vi "DAC Run.vi"(8 "error in":errorcluster, 11 "DAC HS Vib in":refnum<class "DAC HS Vib.lvclass">) -> (0 "error out":errorcluster, 3 "DAC HS Vib out":refnum<class "DAC HS Vib.lvclass">)   [LabVIEW 2019, in "DAC.lvlib" / "DAC HS Vib.lvclass"]
uses:
  DAC HS Vib.lvclass
  C:/Users/krio/Documents/LV_Projects/test-stand/App/DAC/DAC.lvclass
  DAC.lvclass/DAC.ctl
  DAC.lvclass
  Results/Results Method.ctl
  Results/Results.lvlib
  Results/DeepU Results/DeepU Results.lvclass
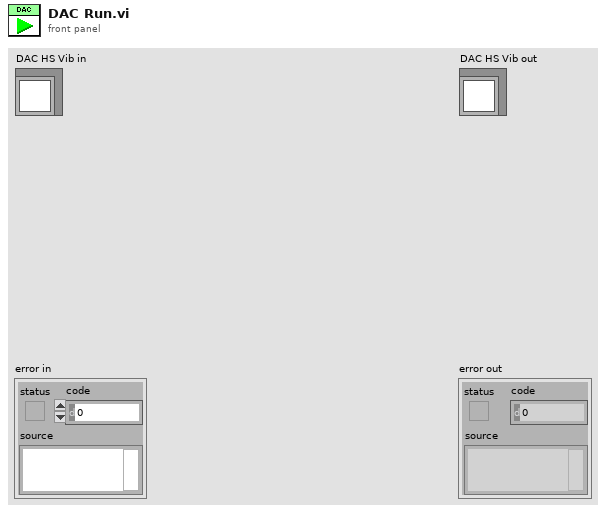
[diagram p1: front panel]
types:
  T1 = typedef "Results.lvlib/Results Method.ctl" = enum16{"Get", "Set"}
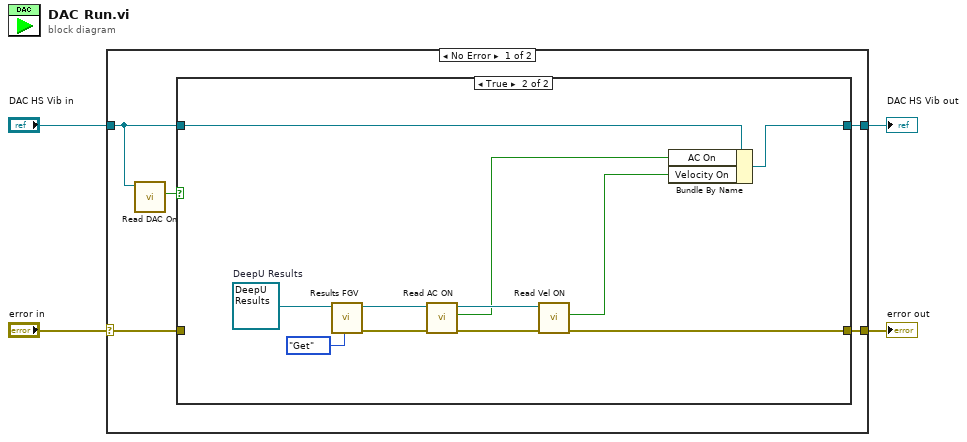
[diagram p0: block diagram]
diagram:
  n1 = case shown="No Error" "error in" {
    selector: "error in" -> [w7 w24]
    tunnel: [w6 w24] -> w2
    tunnel: [w8 w23] -> w1
    tunnel: "DAC HS Vib in" -> [w5 w23]
    frame No Error {
      n2 = call "Read DAC On.vi"("DAC in"=w5) -> ("DAC On"=w9:bool)  [unwired: 8 in, 2 out]
      n3 = case shown="True" w9 {
        tunnel: w5 -> [w11 w22]
        tunnel: [w11 w19] -> w8
        tunnel: w7 -> [w10 _]
        tunnel: [w10 w12] -> w6
        frame False {
        }
        frame True {
          w21 = refnum<class "DeepU Results.lvclass"> refnum  # DeepU Results
          n4 = call-dynamic "Results FGV.vi"("Method"=Results_Method."Get", "DeepU Results in"=w21) -> ("error out"=w14:errorcluster, "DeepU Results out"=w18:refnum<class "DeepU Results.lvclass">)  [unwired: 8 in]
          n5 = call "Read AC ON.vi"("error in (no error)"=w14, "DeepU Results in"=w18) -> ("error out"=w13:errorcluster, "AC ON"=w16:bool, "DeepU Results out"=w17:refnum<class "DeepU Results.lvclass">)  [unwired: 7 in]
          n6 = call "Read Vel ON.vi"("error in (no error)"=w13, "DeepU Results in"=w17) -> ("error out"=w12:errorcluster, "Vel ON"=w15:bool)  [unwired: 7 in, 1 out]
          n7 = Bundle By Name(cluster=w22, "AC On"=w16, "Velocity On"=w15) -> (w19:refnum<class "DAC HS Vib.lvclass">)
        }
      }
    }
    frame Error {
    }
  }
  "error out" <- w2
  "DAC HS Vib out" <- w1
